vi "SngJntArmSim_UpdateX.vi"(8 "dT_Seconds":dbl=0.02, 9 "U":T4, 10 "current_xHat":T4, 11 "SINGLE_JOINT_ARM_SIM":T1 {"GearBox"."Jr_KgM2" format="%13.5p"; "GearBox"."L_H" format="%13.5p"; "GearBox"."Kt_NMPerAmp" format="%13.5p"; "GearBox"."KvINV_RadPerSecPerVolt" format="%13.5p"; "GearBox"."R_Ohms" format="%13.5p"; "GearBox"."FreeSpeed_RadPerSec" format="%13.5p"; "GearBox"."FreeCurrent_Amps" format="%13.5p"; "GearBox"."StallCurrent_Amps" format="%13.5p"; "GearBox"."StallTorque_NM" format="%13.5p"; "GearBox"."nominalVoltage_Volts" format="%13.5p"}) -> (0 "Error":bool, 3 "updated_xHat":T4)   [LabVIEW 2019, in "Trajectory_Library.lvlib"]
doc: "Updates the state of the arm.\n \nInputs:\n - currentXhat -- The current state estimate.\n - u -- The system inputs (voltage).\n - dtSeconds -- The time difference between controller updates.\n\nOutputs:\n - updated_Xhat -- Updated current state estimate\n - error -- If TRUE, an error occured."
uses:
  Trajectory_Library.lvlib
  <vilib>/Analysis/Matrix/Datatypes/RealMatrix.ctl
  TypeDef/SINGLE_JOINT_ARM_SIM.ctl
  TypeDef/LINEAR_SYSTEM_SIM.ctl
  TypeDef/LINEAR_SYSTEM.ctl
  TypeDef/DCMOTOR.CTL
  MatBuilder_Create.vi
  <vilib>/Analysis/Matrix/NI_Matrix.lvlib
panel:
  # "<States, 1>"
  # "<Outputs, 1>"
  # "<Inputs, 1>"
  # "<Outputs, 1>"
  # "<States,States>"
  # "<States,Inputs>"
  # "<Outputs,States>"
  # "<Outputs,Inputs>"
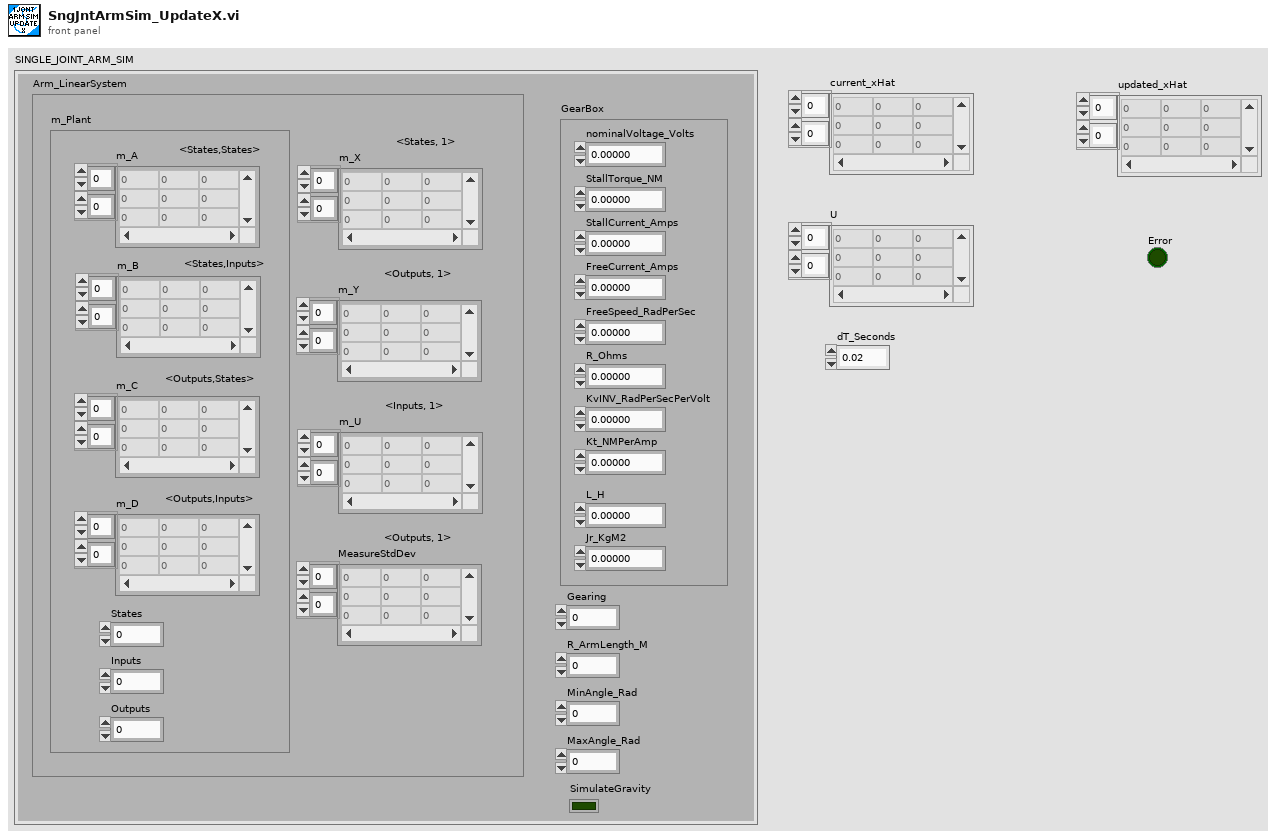
[diagram p1: front panel]
types:
  T1 = typedef "Trajectory_Library.lvlib/SINGLE_JOINT_ARM_SIM.ctl" = cluster{"Arm_LinearSystem":T2, "GearBox":T5, "Gearing":dbl, "R_ArmLength_M":dbl, "MinAngle_Rad":dbl, "MaxAngle_Rad":dbl, "SimulateGravity":bool}
  T2 = typedef "Trajectory_Library.lvlib/LINEAR_SYSTEM_SIM.ctl" = cluster{"m_Plant":T3, "m_X":T4, "m_Y":T4, "m_U":T4, "MeasureStdDev":T4}
  T3 = typedef "Trajectory_Library.lvlib/LINEAR_SYSTEM.ctl" = cluster{"m_A":T4, "m_B":T4, "m_C":T4, "m_D":T4, "States":i32, "Inputs":i32, "Outputs":i32}
  T4 = typedef "NI_Matrix.lvlib/RealMatrix.ctl" = dbl[][]
  T5 = typedef "Trajectory_Library.lvlib/DCMOTOR.CTL" = cluster{"nominalVoltage_Volts":dbl, "StallTorque_NM":dbl, "StallCurrent_Amps":dbl, "FreeCurrent_Amps":dbl, "FreeSpeed_RadPerSec":dbl, "R_Ohms":dbl, "KvINV_RadPerSecPerVolt":dbl, "Kt_NMPerAmp":dbl, "L_H":dbl, "Jr_KgM2":dbl}
  T6 = cluster{"m_A":T4, "m_B":T4, "R_ArmLength_M":dbl, "SimulateGravity":bool}
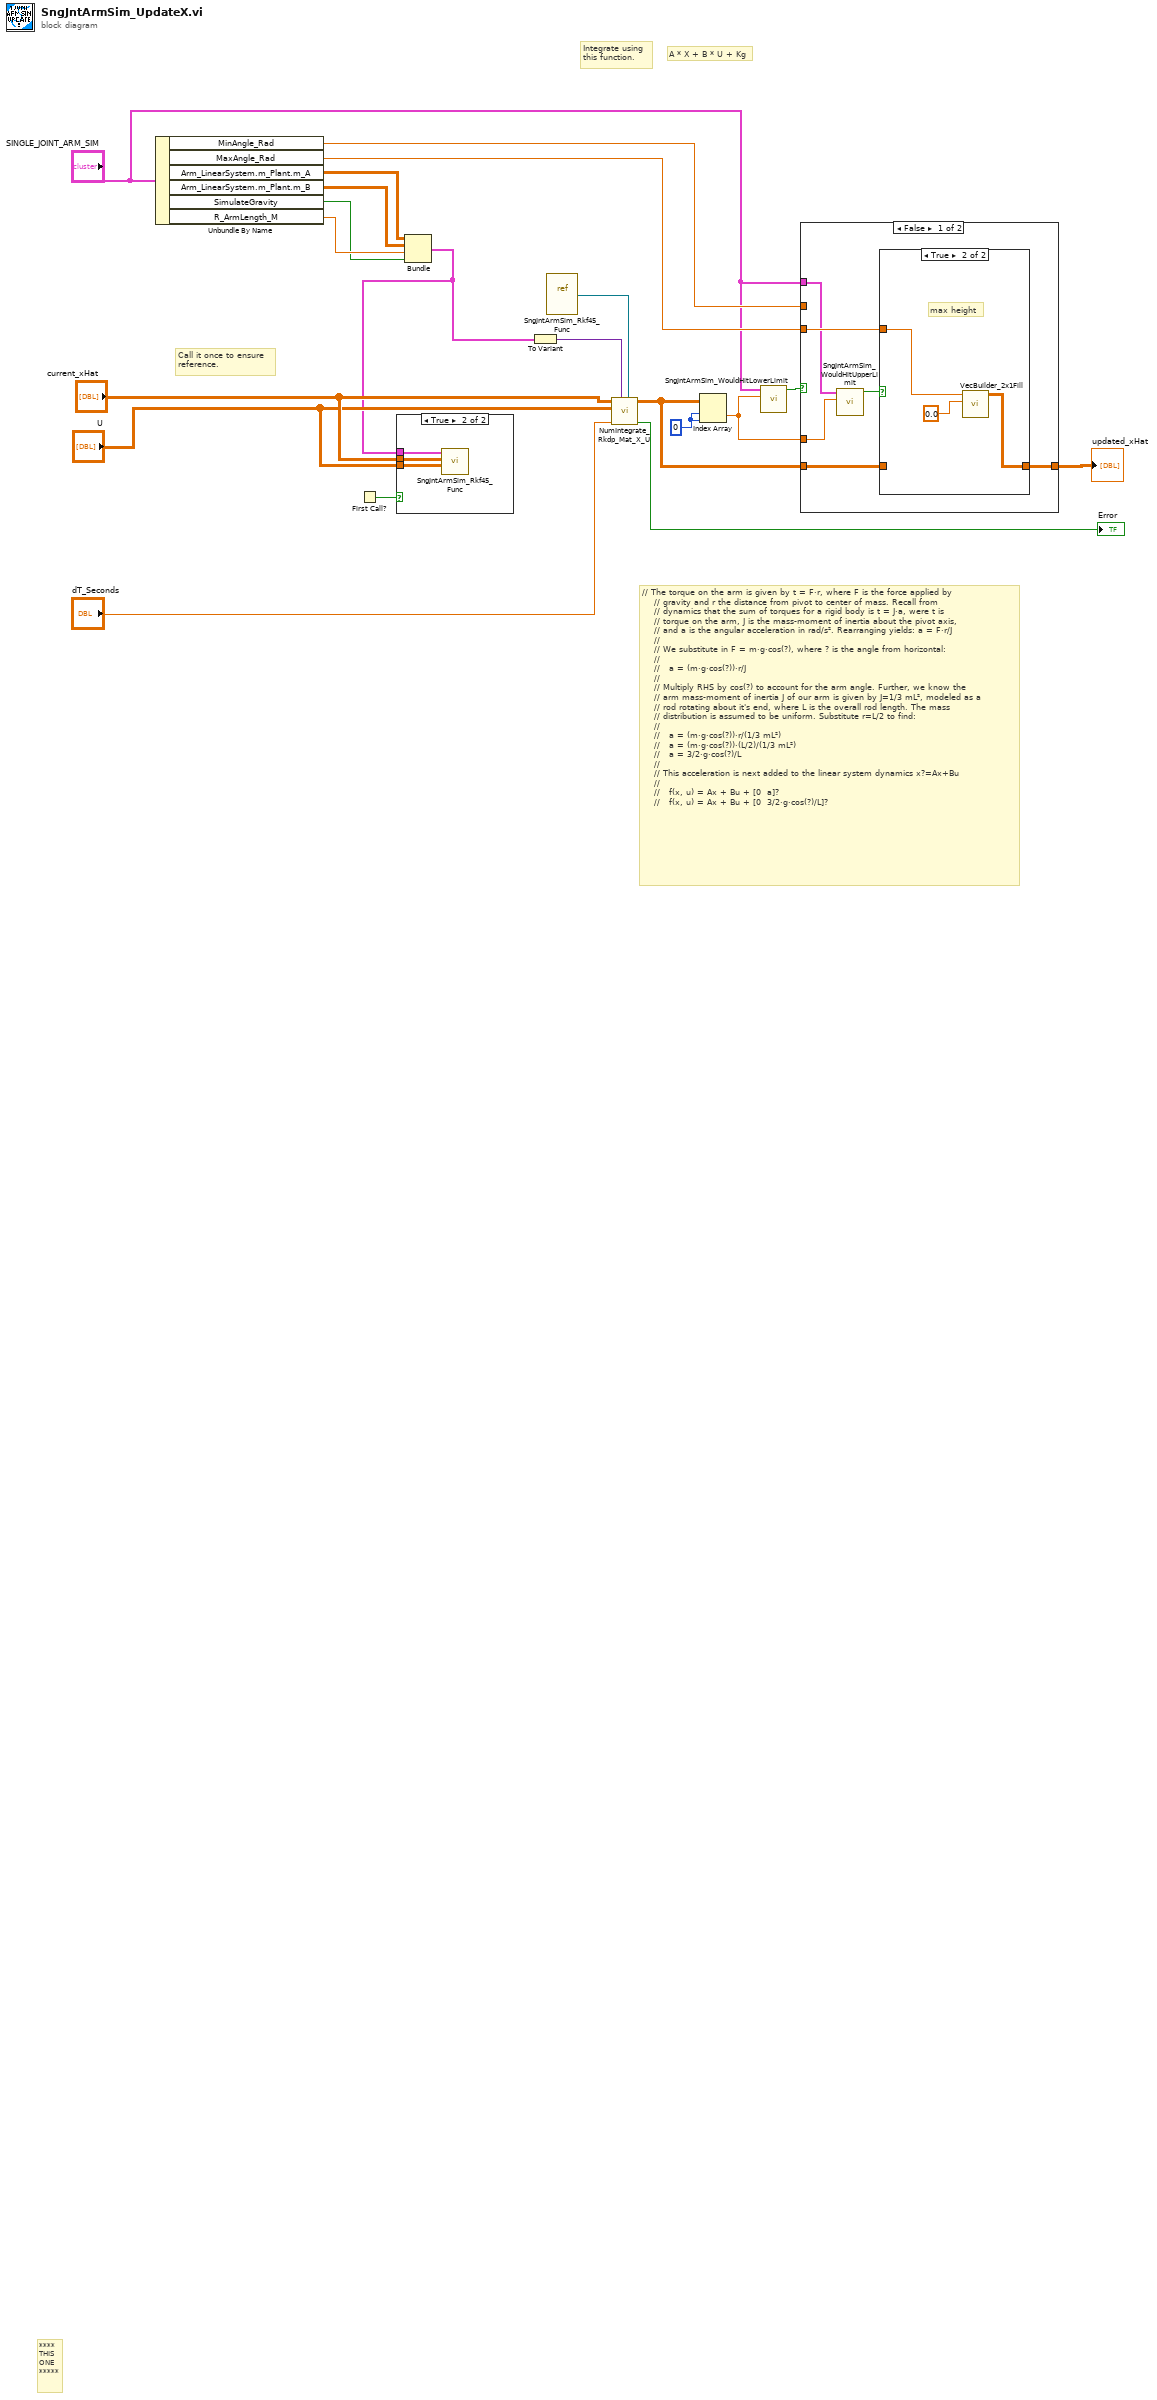
[diagram p0: block diagram]
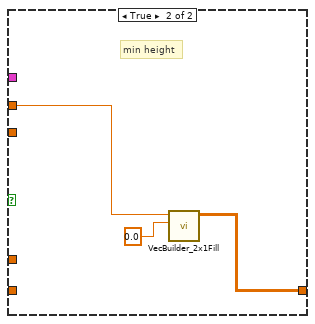
[diagram p4: hidden frame]
diagram:
  w19 = 0 ("index (row)")
  # "// The torque on the arm is given by t = F·r, where F is the force applied by\n    // gravity and r the distance from pivot to center of mass. Recall from\n    // dynamics that the sum of torques for a rigid body is t = J·a, were t is\n    // torque on the arm, J is the mass-moment of inertia about the pivot axis,\n    // and a is the angular acceleration in rad/s². Rearranging yields: a = F·r/J\n    //\n    // We substitute in F = m·g·cos(?), where ? is the angle from horizontal:\n    //\n    //   a = (m·g·cos(?))·r/J\n    //\n    // Multiply RHS by cos(?) to account for the arm angle. Further, we know the\n    // arm mass-moment of inertia J of our arm is given by J=1/3 mL², modeled as a\n    // rod rotating about it's end, where L is the overall rod length. The mass\n    // distribution is assumed to be uniform. Substitute r=L/2 to find:\n    //\n    //   a = (m·g·cos(?))·r/(1/3 mL²)\n    //   a = (m·g·cos(?))·(L/2)/(1/3 mL²)\n    //   a = 3/2·g·cos(?)/L\n    //\n    // This acceleration is next added to the linear system dynamics x?=Ax+Bu\n    //\n    //   f(x, u) = Ax + Bu + [0  a]?\n    //   f(x, u) = Ax + Bu + [0  3/2·g·cos(?)/L]?"
  # "Call it once to ensure\nreference."
  # "Integrate using\nthis function."
  # "A * X + B * U + Kg"
  # "****\nTHIS\nONE\n*****"
  n1 = Unbundle By Name("SINGLE_JOINT_ARM_SIM") -> ("MinAngle_Rad"=w13:dbl, "MaxAngle_Rad"=w18:dbl, "Arm_LinearSystem.m_Plant.m_A"=w11:T4, "Arm_LinearSystem.m_Plant.m_B"=w10:T4, "SimulateGravity"=w8:bool, "R_ArmLength_M"=w9:dbl)
  n2 = First Call?() -> (First Call?: T/F=w4:bool)
  n3 = Bundle("m_A"=w11, "m_B"=w10, "R_ArmLength_M"=w9, "SimulateGravity"=w8) -> (w2:T6)  [unwired: 1 in]
  n4 = case shown="True" w4 {
    tunnel: "current_xHat" -> [_ w23]
    tunnel: "U" -> [_ w22]
    tunnel: w2 -> [_ w21]
    frame False {
    }
    frame True {
      n5 = call "SngJntArmSim_Rkf45_Func.vi"("U"=w22, "X"=w23, "Variant"=w21) -> ()  [unwired: 7 in, 2 out]
    }
  }
  n6 = To Variant(anything=w2) -> (Variant=w1:variant)
  n7 = vi-ref "SngJntArmSim_Rkf45_Func.vi"() -> (w5:refnum<vi>)
  n8 = call "NumIntegrate_Rkdp_Mat_X_U.vi"("Func_X_U_Extra"=w5, "PassedData"=w1, "dT_Seconds"="dT_Seconds", "U"="U", "X"="current_xHat") -> ("Error"=→"Error":bool, "Return X"=w17:T4)  [unwired: 4 in, 1 out]
  n9 = Index Array(array=w17, index (row)=w19, index (col)=w19) -> (element=w14:dbl)
  n10 = call "SngJntArmSim_WouldHitLowerLimit.vi"("Angle_Rads"=w14, "SingleJointArmSim"="SINGLE_JOINT_ARM_SIM") -> ("WouldHitLowLimit"=w15:bool)  [unwired: 9 in]
  n11 = case shown="False" w15 {
    tunnel: w18 -> [w25 _]
    tunnel: w17 -> [w29 _]
    tunnel: [w28 w34] -> w16
    tunnel: w14 -> [w26 _]
    tunnel: w13 -> [_ w35]
    tunnel: "SINGLE_JOINT_ARM_SIM" -> [w24 _]
    frame False {
      n12 = call "SngJntArmSim_WouldHitUpperLimit.vi"("Angle_Rad"=w26, "SingleJointArmSim"=w24) -> ("Would Hit HIgh LImit"=w27:bool)  [unwired: 9 in]
      n13 = case shown="True" w27 {
        tunnel: w29 -> [w30 _]
        tunnel: [w30 w31] -> w28
        tunnel: w25 -> [_ w32]
        frame False {
        }
        frame True {
          # "max height"
          n14 = call "VecBuilder_2x1Fill.vi"("R1"=0.0, "R0"=w32) -> ("output matrix"=w31:T4)  [unwired: 9 in]
        }
      }
    }
    frame True {
      # "min height"
      n15 = call "VecBuilder_2x1Fill.vi"("R1"=0.0, "R0"=w35) -> ("output matrix"=w34:T4)  [unwired: 9 in]
    }
  }
  "updated_xHat" <- w16
